vi "read.vi"(3 "X/Y":bool, 5 "VISA resource name":refnum<visa-resource-name> caption="VISA资源名称") -> (0 "错误输出":errorcluster, 1 "电机位置":u32, 2 "读取缓冲区":string)   [LabVIEW 2020]
uses:
  <vilib>/Instr/_visa.llb/VISA Configure Serial Port (Instr).vi
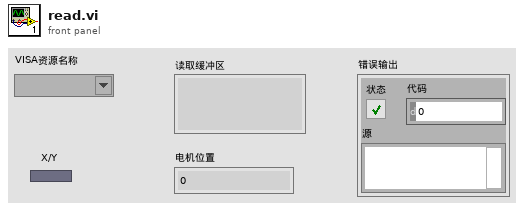
[diagram p1: front panel]
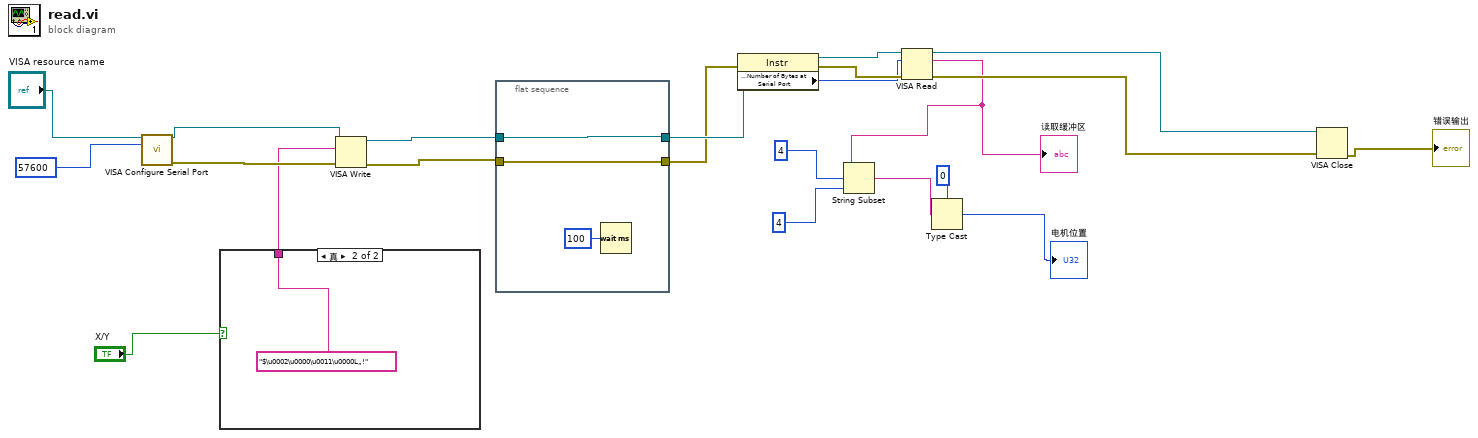
[diagram p0: block diagram]
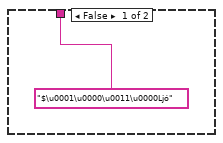
[diagram p2: hidden frame]
diagram:
  n1 = call-poly "VISA Configure Serial Port"("VISA resource name"="VISA resource name", "baud rate (9600)"=u32 57600) -> ("VISA resource name out"=w22:refnum<visa-resource-name>, "error out"=w21:errorcluster)  [unwired: 12 in]
  n2 = case shown="真" "X/Y" {
    tunnel: ["$\u0001\u0000\u0011\u0000Ljó" ("写入缓冲区") "$\u0002\u0000\u0011\u0000L„!" ("写入缓冲区")] -> w13
    frame False {
    }
    frame True {
    }
  }
  n3 = VISA Write(VISA resource name=w22, write buffer=w13, error in (no error)=w21) -> (VISA resource name out=w15:refnum<visa-resource-name>, error out=w14:errorcluster)  [unwired: 1 out]
  n4 = flat-sequence {
    tunnel: w15 -> [w26]
    tunnel: [w26] -> w12
    tunnel: w14 -> [w25]
    tunnel: [w25] -> w11
    frame #0 {
      n5 = Wait (ms)(milliseconds to wait=u32 100 ("等待时间（毫秒）")) -> ()  [unwired: 1 out]
    }
  }
  n6 = property class="Instr"(reference=w12, error in=w11) -> (reference out=w10:refnum<visa-resource-name>, error out=w9:errorcluster, "Serial Settings:Number of Bytes at Serial Port"=w8:u32)
  n7 = VISA Read(VISA resource name=w10, byte count=w8, error in (no error)=w9) -> (VISA resource name out=w18:refnum<visa-resource-name>, read buffer=w7:string, error out=w17:errorcluster)  [unwired: 1 out]
  "读取缓冲区" <- w7
  n8 = String Subset(string=w7, offset (0)=4 ("偏移量(0)"), length (rest)=4 ("长度（剩余）")) -> (substring=w4:string)
  n9 = Type Cast(type=u32 0, x=w4) -> (*(type *) &x=→"电机位置":u32)
  n10 = VISA Close(VISA resource name=w18, error in (no error)=w17) -> (error out=→"错误输出":errorcluster)
